vi "Pasopaso.vi"() -> ()   [LabVIEW 2023]
uses:
  <vilib>/Instr/_visa.llb/VISA Configure Serial Port (Instr).vi
panel:
  in  "ACTIVA 2":bool caption="ACTIVA"
  in  "ACTIVA":bool
  in  "VELOCIDAD2":dbl(knob)=91.94641936786925 caption="VELOCIDAD" scale=0.0..100.0
  in  "PARAR 2":bool
  in  "Izquierda 2":bool
  in  "Derecha 2":bool
  in  "PASOS2":dbl=5.0 caption="PASOS"
  in  "VELOCIDAD1":dbl(knob)=91.94641936786925 caption="VELOCIDAD" scale=0.0..100.0
  in  "PARAR":bool
  in  "Izquierda":bool
  in  "Derecha":bool
  in  "PASOS":dbl=5.0
  in  "PUERTO":refnum<visa-resource-name>="COM4"
  in  "stop":bool
  # "MOTOR1"
  # "MOTOR2"
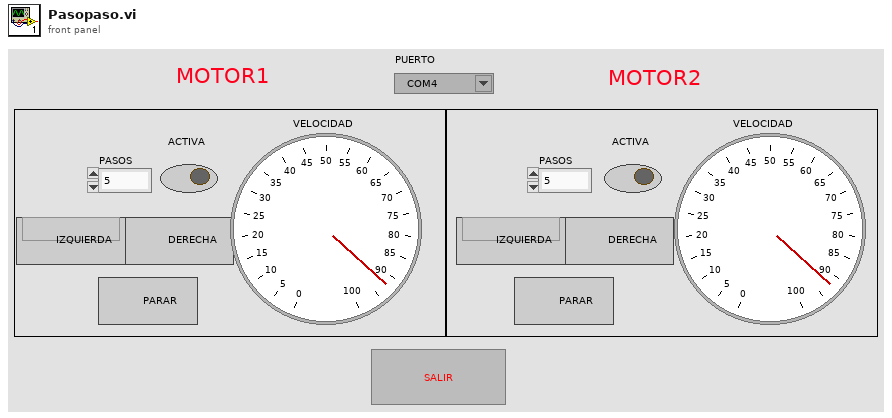
[diagram p1: front panel]
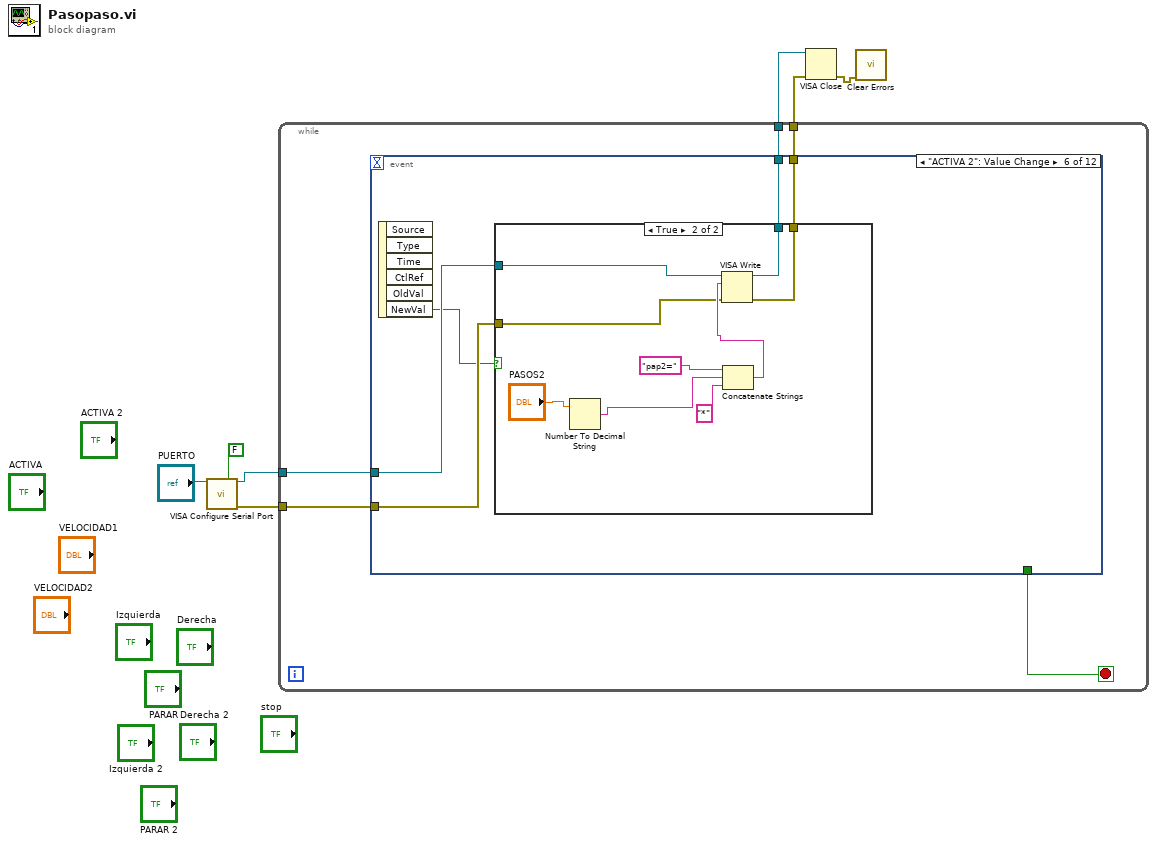
[diagram p0: block diagram]
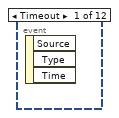
[diagram p2: hidden frame]
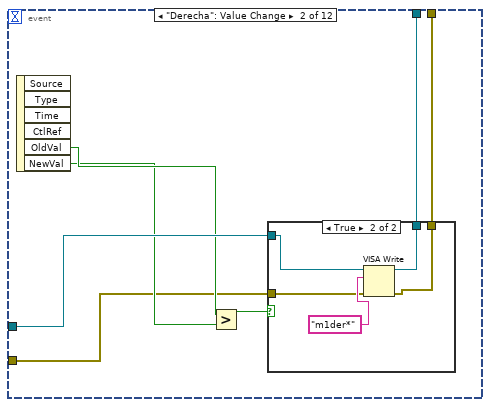
[diagram p3: hidden frame]
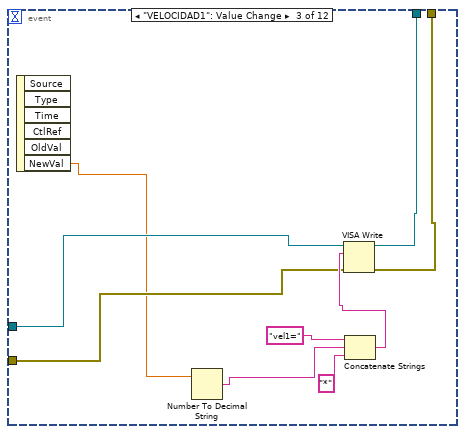
[diagram p5: hidden frame]
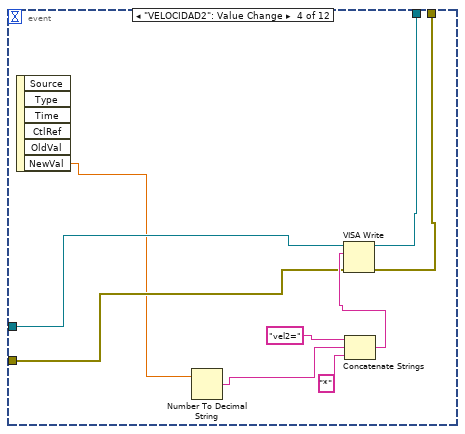
[diagram p6: hidden frame]
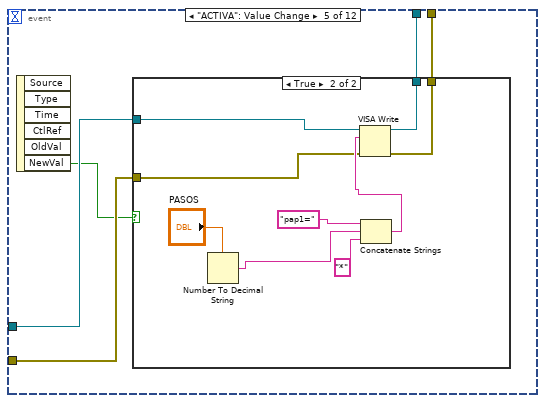
[diagram p7: hidden frame]
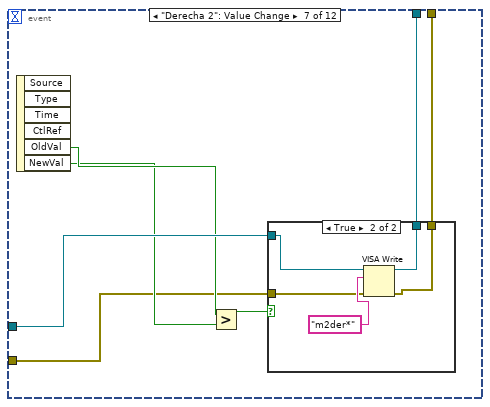
[diagram p10: hidden frame]
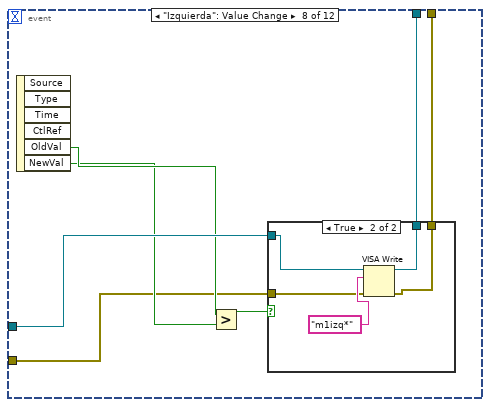
[diagram p12: hidden frame]
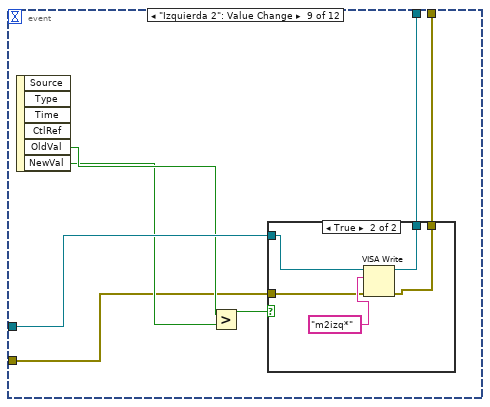
[diagram p14: hidden frame]
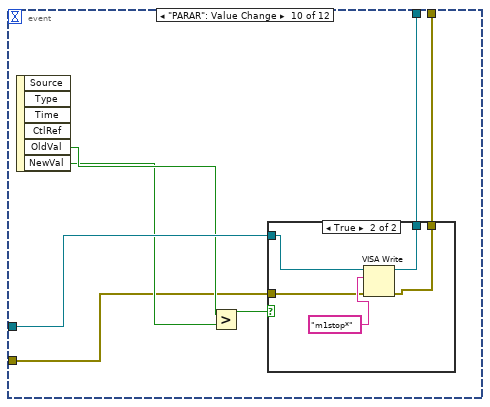
[diagram p16: hidden frame]
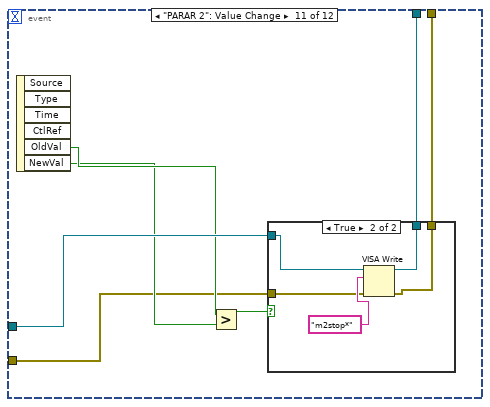
[diagram p18: hidden frame]
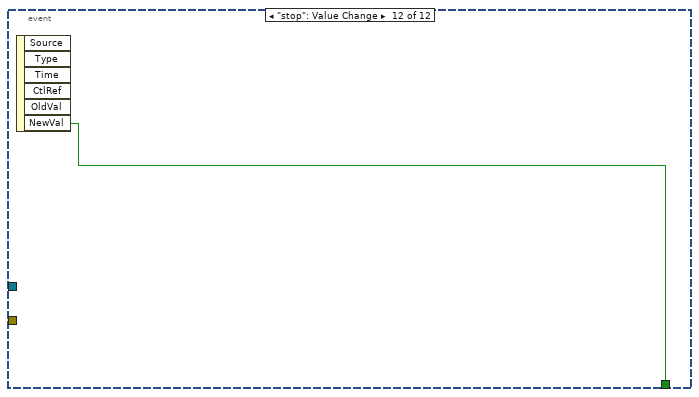
[diagram p20: hidden frame]
diagram:
  n1 = call-poly "VISA Configure Serial Port"("VISA resource name"="PUERTO", "Enable Termination\nChar (T)"=FALSE ("Enable Termination\nChar (T)")) -> ("VISA resource name out"=w4:refnum<visa-resource-name>, "error out"=w3:errorcluster)  [unwired: 12 in]
  n2 = while {
    tunnel: w4 -> [w12]
    tunnel: w3 -> [w11]
    tunnel: [w10] -> w2
    tunnel: [w9] -> w1
    stop <- w8 stop-if-true
    n3 = event shown="[5] \"ACTIVA 2\": Value Change" {
      selector: _ -> [_ _ _ _ _ _ _ _ _ _ _ _]
      dyn-events: _ -> [_ _ _ _ _ _ _ _ _ _ _ _]
      timeout: _ -> [_ _ _ _ _ _ _ _ _ _ _ _]
      tunnel: w12 -> [_ w19 w29 w38 w47 w61 w77 w89 w101 w113 w125 _]
      tunnel: w11 -> [_ w15 w28 w37 w46 w60 w73 w85 w97 w109 w121 _]
      tunnel: [_ w14 w26 w35 w44 w58 w72 w84 w96 w108 w120 _] -> w10
      tunnel: [_ w13 w27 w36 w45 w59 w71 w83 w95 w107 w119 _] -> w9
      tunnel: [_ _ _ _ _ _ _ _ _ _ _ w131] -> w8
      event Timeout {
        n4 = event-data() -> ()  [unwired: 1 in, 3 out]
      }
      event "Derecha": Value Change {
        n5 = event-data() -> ("OldVal"=w18:bool, "NewVal"=w17:bool)  [unwired: 1 in, 4 out]
        n6 = Greater?(x=w18, y=w17) -> (0:w16:bool)
        n7 = case shown="True" w16 {
          tunnel: w19 -> [_ w24]
          tunnel: [_ w23] -> w14
          tunnel: w15 -> [_ w21]
          tunnel: [_ w20] -> w13
          frame False {
          }
          frame True {
            n8 = VISA Write(VISA resource name=w24, write buffer="m1der*", error in (no error)=w21) -> (VISA resource name out=w23:refnum<visa-resource-name>, error out=w20:errorcluster)  [unwired: 1 out]
          }
        }
      }
      event "VELOCIDAD1": Value Change {
        n9 = event-data() -> ("NewVal"=w25:dbl)  [unwired: 1 in, 5 out]
        n10 = Number To Decimal String(number=w25) -> (decimal integer string=w32:string)  [unwired: 1 in]
        n11 = Concatenate Strings("vel1=" ("string"), w32, "*" ("string")) -> (w30:string)
        n12 = VISA Write(VISA resource name=w29, write buffer=w30, error in (no error)=w28) -> (VISA resource name out=w26:refnum<visa-resource-name>, error out=w27:errorcluster)  [unwired: 1 out]
      }
      event "VELOCIDAD2": Value Change {
        n13 = event-data() -> ("NewVal"=w34:dbl)  [unwired: 1 in, 5 out]
        n14 = Number To Decimal String(number=w34) -> (decimal integer string=w41:string)  [unwired: 1 in]
        n15 = Concatenate Strings("vel2=" ("string"), w41, "*" ("string")) -> (w39:string)
        n16 = VISA Write(VISA resource name=w38, write buffer=w39, error in (no error)=w37) -> (VISA resource name out=w35:refnum<visa-resource-name>, error out=w36:errorcluster)  [unwired: 1 out]
      }
      event "ACTIVA": Value Change {
        n17 = event-data() -> ("NewVal"=w43:bool)  [unwired: 1 in, 5 out]
        n18 = case shown="True" w43 {
          tunnel: w47 -> [_ w52]
          tunnel: w46 -> [_ w51]
          tunnel: [_ w50] -> w45
          tunnel: [_ w49] -> w44
          frame False {
          }
          frame True {
            n19 = Number To Decimal String(number="PASOS") -> (decimal integer string=w55:string)  [unwired: 1 in]
            n20 = Concatenate Strings("pap1=" ("string"), w55, "*" ("string")) -> (w53:string)
            n21 = VISA Write(VISA resource name=w52, write buffer=w53, error in (no error)=w51) -> (VISA resource name out=w49:refnum<visa-resource-name>, error out=w50:errorcluster)  [unwired: 1 out]
          }
        }
      }
      event "ACTIVA 2": Value Change {
        n22 = event-data() -> ("NewVal"=w57:bool)  [unwired: 1 in, 5 out]
        n23 = case shown="True" w57 {
          tunnel: w61 -> [_ w66]
          tunnel: w60 -> [_ w65]
          tunnel: [_ w64] -> w59
          tunnel: [_ w63] -> w58
          frame False {
          }
          frame True {
            n24 = Number To Decimal String(number="PASOS2") -> (decimal integer string=w69:string)  [unwired: 1 in]
            n25 = Concatenate Strings("pap2=" ("string"), w69, "*" ("string")) -> (w67:string)
            n26 = VISA Write(VISA resource name=w66, write buffer=w67, error in (no error)=w65) -> (VISA resource name out=w63:refnum<visa-resource-name>, error out=w64:errorcluster)  [unwired: 1 out]
          }
        }
      }
      event "Derecha 2": Value Change {
        n27 = event-data() -> ("OldVal"=w76:bool, "NewVal"=w75:bool)  [unwired: 1 in, 4 out]
        n28 = Greater?(x=w76, y=w75) -> (0:w74:bool)
        n29 = case shown="True" w74 {
          tunnel: w77 -> [_ w82]
          tunnel: [_ w81] -> w72
          tunnel: w73 -> [_ w79]
          tunnel: [_ w78] -> w71
          frame False {
          }
          frame True {
            n30 = VISA Write(VISA resource name=w82, write buffer="m2der*", error in (no error)=w79) -> (VISA resource name out=w81:refnum<visa-resource-name>, error out=w78:errorcluster)  [unwired: 1 out]
          }
        }
      }
      event "Izquierda": Value Change {
        n31 = event-data() -> ("OldVal"=w88:bool, "NewVal"=w87:bool)  [unwired: 1 in, 4 out]
        n32 = Greater?(x=w88, y=w87) -> (0:w86:bool)
        n33 = case shown="True" w86 {
          tunnel: w89 -> [_ w94]
          tunnel: [_ w93] -> w84
          tunnel: w85 -> [_ w91]
          tunnel: [_ w90] -> w83
          frame False {
          }
          frame True {
            n34 = VISA Write(VISA resource name=w94, write buffer="m1izq*", error in (no error)=w91) -> (VISA resource name out=w93:refnum<visa-resource-name>, error out=w90:errorcluster)  [unwired: 1 out]
          }
        }
      }
      event "Izquierda 2": Value Change {
        n35 = event-data() -> ("OldVal"=w100:bool, "NewVal"=w99:bool)  [unwired: 1 in, 4 out]
        n36 = Greater?(x=w100, y=w99) -> (0:w98:bool)
        n37 = case shown="True" w98 {
          tunnel: w101 -> [_ w106]
          tunnel: [_ w105] -> w96
          tunnel: w97 -> [_ w103]
          tunnel: [_ w102] -> w95
          frame False {
          }
          frame True {
            n38 = VISA Write(VISA resource name=w106, write buffer="m2izq*", error in (no error)=w103) -> (VISA resource name out=w105:refnum<visa-resource-name>, error out=w102:errorcluster)  [unwired: 1 out]
          }
        }
      }
      event "PARAR": Value Change {
        n39 = event-data() -> ("OldVal"=w112:bool, "NewVal"=w111:bool)  [unwired: 1 in, 4 out]
        n40 = Greater?(x=w112, y=w111) -> (0:w110:bool)
        n41 = case shown="True" w110 {
          tunnel: w113 -> [_ w118]
          tunnel: [_ w117] -> w108
          tunnel: w109 -> [_ w115]
          tunnel: [_ w114] -> w107
          frame False {
          }
          frame True {
            n42 = VISA Write(VISA resource name=w118, write buffer="m1stop*", error in (no error)=w115) -> (VISA resource name out=w117:refnum<visa-resource-name>, error out=w114:errorcluster)  [unwired: 1 out]
          }
        }
      }
      event "PARAR 2": Value Change {
        n43 = event-data() -> ("OldVal"=w124:bool, "NewVal"=w123:bool)  [unwired: 1 in, 4 out]
        n44 = Greater?(x=w124, y=w123) -> (0:w122:bool)
        n45 = case shown="True" w122 {
          tunnel: w125 -> [_ w130]
          tunnel: [_ w129] -> w120
          tunnel: w121 -> [_ w127]
          tunnel: [_ w126] -> w119
          frame False {
          }
          frame True {
            n46 = VISA Write(VISA resource name=w130, write buffer="m2stop*", error in (no error)=w127) -> (VISA resource name out=w129:refnum<visa-resource-name>, error out=w126:errorcluster)  [unwired: 1 out]
          }
        }
      }
      event "stop": Value Change {
        n47 = event-data() -> ("NewVal"=w131:bool)  [unwired: 1 in, 5 out]
      }
    }
  }
  n48 = VISA Close(VISA resource name=w2, error in (no error)=w1) -> (error out=w5:errorcluster)
  n49 = call <vilib>:"Clear Errors.vi"("error in (no error)"=w5) -> ()  [unwired: 5 in, 2 out]
